vi "RemoteVI Apply Splitter.vi"(0 "VI":refnum<vi>, 1 "hWnd":u64, 2 "bars":T1(array[cluster]), 3 "busy?":bool) -> (4 "moved?":bool)   [LabVIEW 2020, in "RemoteVI.lvlib"]
doc: "Moves a splitter bar a client dragged (s id pos, docs\\protocol.md section 4) - LabVIEW moves a splitter bar only while it tracks the real mouse, which the server never moves, so the bar is set through VI Server instead. Only while busy? is FALSE (no popup and no modal window is open: a VI Server call would block in their modal loop), the move stored for hWnd is taken from RemoteVI Splitter Request.vi; while busy it stays stored. The bar is element id of {LV.Panel} Splitters[] of VI's panel; bars (RemoteVI Read Splitters.vi) says where its edge is in the frame, so its {LV.Splitter} Position becomes Position + (pos - edge), with edge the bar's x for a vertical bar and y for a horizontal one. LabVIEW keeps its own minimum pane sizes. An id that is no bar of bars does nothing. moved? is TRUE when a Position was written without error; the server loop then reads the bars, tips and origin again."
uses:
  RemoteVI.lvlib
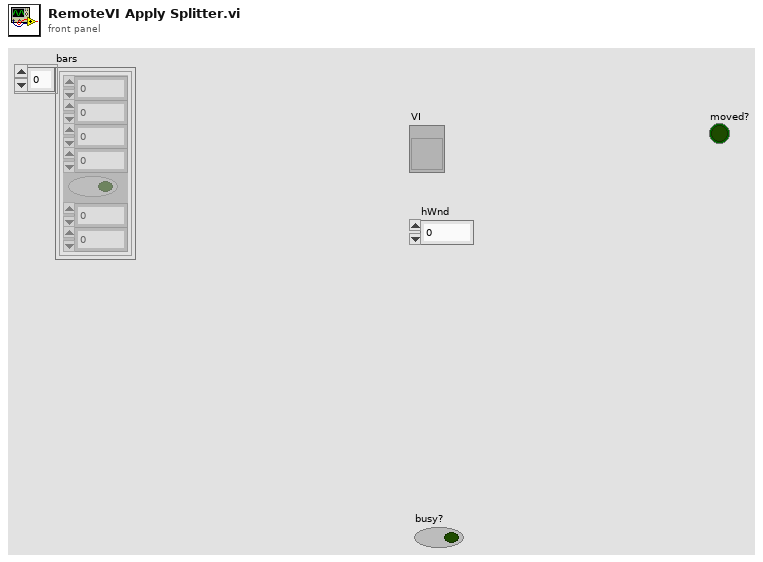
[diagram p1: front panel]
types:
  T1 = cluster{"x":i32, "y":i32, "w":i32, "h":i32, "vertical":bool, "min":i32, "max":i32}[]
  T2 = cluster{"x":i32, "y":i32, "w":i32, "h":i32, "vertical":bool, "min":i32, "max":i32}
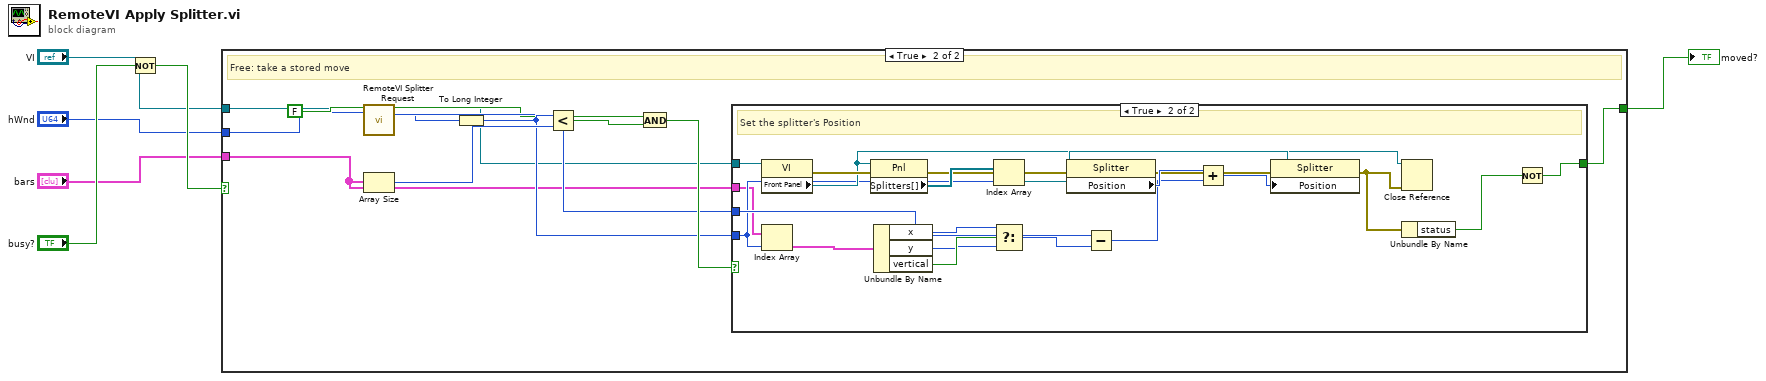
[diagram p0: block diagram]
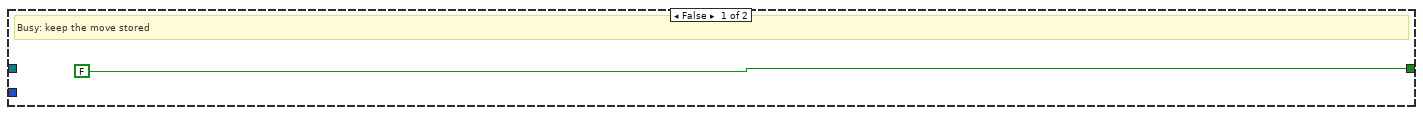
[diagram p2: hidden frame]
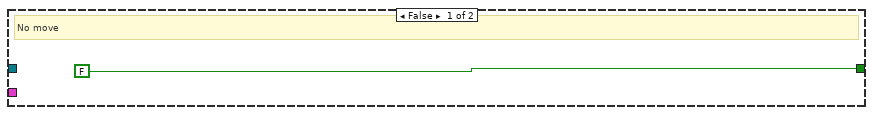
[diagram p3: hidden frame]
diagram:
  n1 = Not(x="busy?") -> (.not. x?=w5:bool)
  n2 = case shown="True" w5 {
    tunnel: "VI" -> [_ w8]
    tunnel: "hWnd" -> [_ w9]
    tunnel: "bars" -> [_ w10]
    tunnel: [FALSE w19] -> w6
    frame False {
      # "Busy: keep the move stored"
    }
    frame True {
      # "Free: take a stored move"
      n3 = call "RemoteVI Splitter Request.vi"("put?"=FALSE, "hWnd"=w9) -> ("pending?"=w12:bool, "id out"=w13:u64, "pos out"=w14:i32)  [unwired: 11 in]
      n4 = Array Size(array=w10) -> (size(s)=w16:i32)
      n5 = To Long Integer(number=w13) -> (32bit integer=w15:i32)
      n6 = Less?(x=w15, y=w16) -> (x < y?=w17:bool)
      n7 = And(x=w12, y=w17) -> (x .and. y?=w18:bool)
      n8 = case shown="True" w18 {
        tunnel: w8 -> [_ w21]
        tunnel: w10 -> [_ w22]
        tunnel: w14 -> [_ w24]
        tunnel: w15 -> [_ w23]
        tunnel: [FALSE w41] -> w19
        frame False {
          # "No move"
        }
        frame True {
          # "Set the splitter's Position"
          n9 = property class="VI"(reference=w21) -> (error out=w32:errorcluster, "Front Panel"=w31:refnum<vi>)  [unwired: 1 in, 1 out]
          n10 = Index Array(array=w22, index=w23) -> (element=w25:T2)
          n11 = property class="Pnl"(reference=w31, error in=w32) -> (error out=w33:errorcluster, "Splitters[]"=w34:refnum<vi>[])  [unwired: 1 out]
          n12 = Unbundle By Name(w25) -> ("x"=w26:i32, "y"=w27:i32, "vertical"=w28:bool)
          n13 = Index Array(array=w34, index=w23) -> (element=w35:refnum<vi>)
          n14 = Select(t=w26, s=w28, f=w27) -> (s? t:f=w29:i32)
          n15 = property class="Splitter"(reference=w35, error in=w33) -> (error out=w36:errorcluster, "Position"=w37:i32)  [unwired: 1 out]
          n16 = Subtract(x=w24, y=w29) -> (x-y=w30:i32)
          n17 = Add(x=w37, y=w30) -> (x+y=w38:i32)
          n18 = property class="Splitter"(reference=w35, error in=w36, "Position"=w38) -> (error out=w39:errorcluster)  [unwired: 1 out]
          n19 = Close Reference(reference=w31, error in (no error)=w39) -> ()  [unwired: 1 out]
          n20 = Unbundle By Name(w39) -> ("status"=w40:bool)
          n21 = Not(x=w40) -> (.not. x?=w41:bool)
        }
      }
    }
  }
  "moved?" <- w6
